vi "VIH HelpGen - FILE - Get Qualified Filename.vi"(11 "File Path":path) -> (0 "File Type":T1, 2 "Qualified name":string)   [LabVIEW 2014]
doc: "::: VI Helpeks :::\nCopyright (c) 2000-2026 Konstantin Shifershteyn. All rights reserved."
uses:
  _VIH HelpGen - Palette.llb/VIH HelpGen Typedef - Palette - Item Type Enum.ctl
panel:
  # "VI Helpeks\nCopyright (c) 2012-2026 Konstantin Shifershteyn"
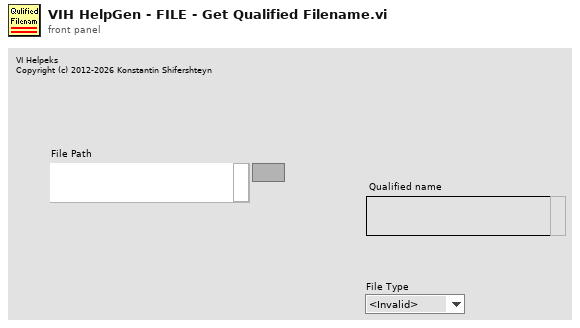
[diagram p1: front panel]
types:
  T1 = typedef "VIH HelpGen Typedef - Palette - Item Type Enum.ctl" = enum32{"<Invalid>", "<unknown>", "VI", "Menu", "LV Func", "Express VI", "Poly VI", "CTL", "HTML"}
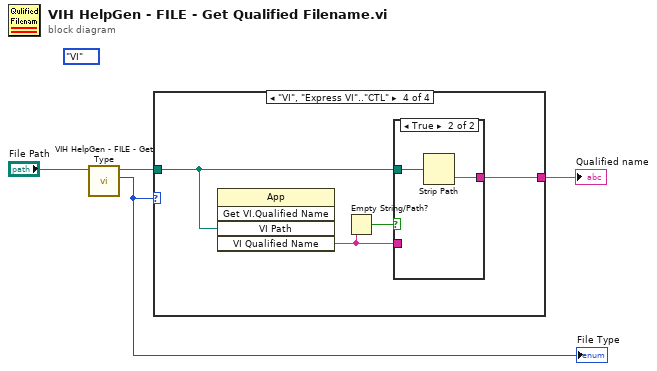
[diagram p0: block diagram]
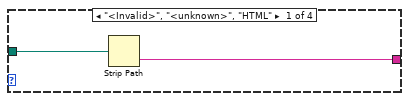
[diagram p2: hidden frame]
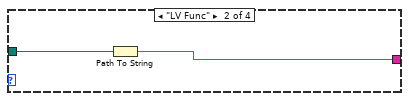
[diagram p3: hidden frame]
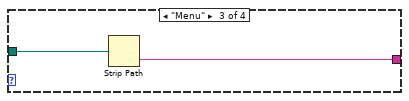
[diagram p4: hidden frame]
diagram:
  (unwired) VIH_HelpGen_Typedef_-_Palette_-_Item_Type_Enum."VI" ("File Type")
  n1 = call "VIH HelpGen - FILE - Get Type.vi"("File Path"="File Path") -> ("File Type"=w1:T1, "dup File Path"=w2:path)  [unwired: 8 in, 1 out]
  "File Type" <- w1
  n2 = case shown="\"VI\", \"Express VI\"..\"CTL\"" w1 {
    tunnel: [w5 w7 w9 w13] -> w4
    tunnel: w2 -> [w6 w8 w10 w11]
    frame "<Invalid>", "<unknown>", "HTML" {
      n3 = Strip Path(path=w6) -> (name=w5:string)  [unwired: 1 out]
    }
    frame "LV Func" {
      n4 = Path To String(path=w8) -> (string=w7:string)
    }
    frame "Menu" {
      n5 = Strip Path(path=w10) -> (name=w9:string)  [unwired: 1 out]
    }
    frame "VI", "Express VI".."CTL" {
      n6 = invoke class="App" method="Get VI.Qualified Name"("VI Path"=w11) -> ("VI Qualified Name"=w12:string)  [unwired: 4 in, 4 out]
      n7 = Empty String/Path?(string/path=w12) -> (empty?=w14:bool)
      n8 = case shown="True" w14 {
        tunnel: [w15 w16] -> w13
        tunnel: w12 -> [w15 _]
        tunnel: w11 -> [_ w17]
        frame False {
        }
        frame True {
          n9 = Strip Path(path=w17) -> (name=w16:string)  [unwired: 1 out]
        }
      }
    }
  }
  "Qualified name" <- w4
